vi "test Remote IO DIO Loop Back.vi"(8 "error in (no error)":errorcluster, 11 "TestCase in":refnum<class "Scan Engine EtherCAT System Tests.lvclass">) -> (0 "error out":errorcluster, 3 "TestCase out":refnum<class "Scan Engine EtherCAT System Tests.lvclass">)   [LabVIEW 2020, in "Scan Engine EtherCAT System Tests.lvclass"]
uses:
  Scan Engine EtherCAT System Tests.lvclass
  C:/Program Files (x86)/National Instruments/LabVIEW 2020/vi.lib/NI/VeriStand Custom Device Testing Tools/VeriStandTestCase/VeriStandTestCase.lvclass
  <vilib>/addons/_JKI Toolkits/VI Tester/TestCase.llb/TestCase.lvclass
  <vilib>/NI/VeriStand Custom Device Testing Tools/VeriStandTestCase/VeriStandTestCase.lvclass
  C:/Program Files (x86)/National Instruments/LabVIEW 2020/vi.lib/addons/_JKI Toolkits/VI Tester/TestCase.llb/TestCase.lvclass
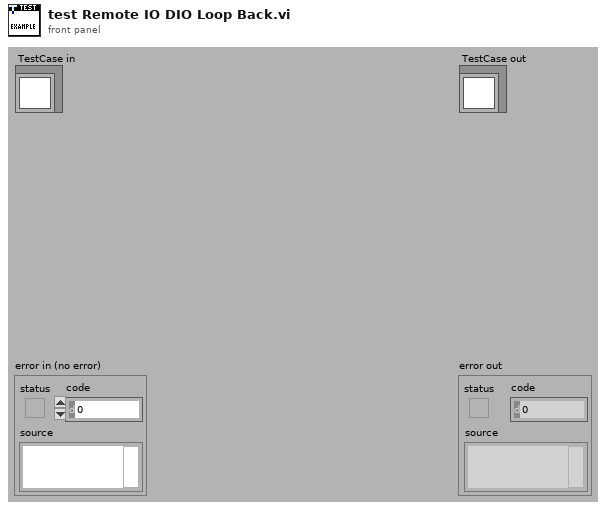
[diagram p1: front panel]
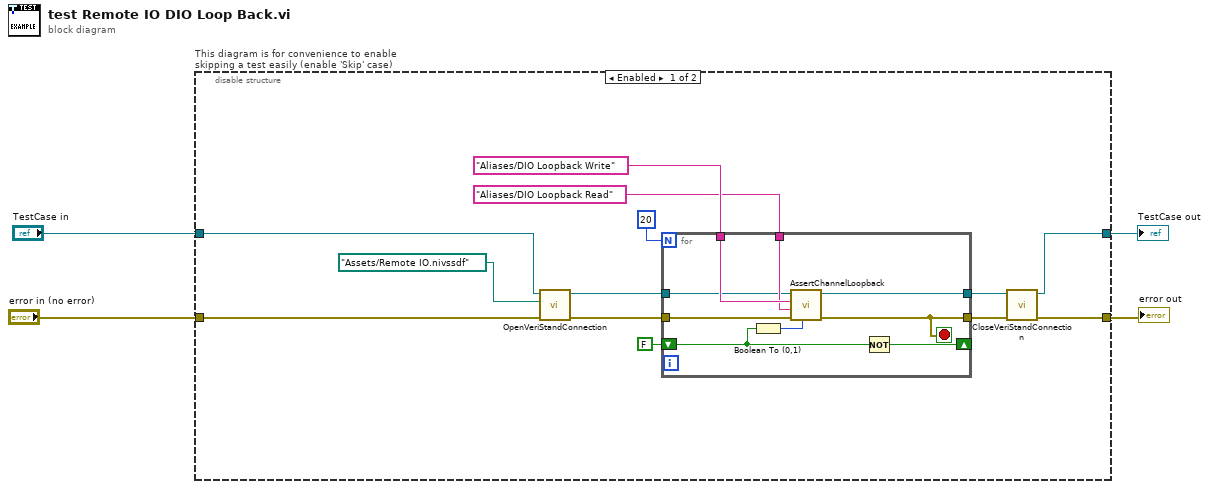
[diagram p0: block diagram]
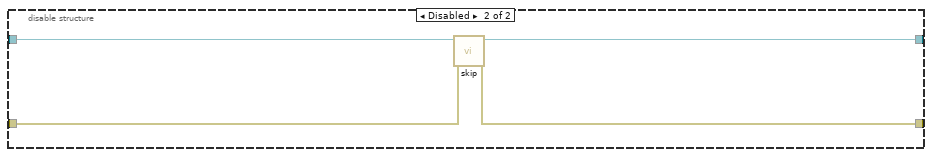
[diagram p2: hidden frame]
diagram:
  n1 = disable-structure "This diagram is for convenience to enable skipping a test easily (enable 'Skip' case)" shown="Enabled" {
    disable-tunnel: "TestCase in" -> [w6 w30]
    disable-tunnel: [w5 w28] -> w1
    disable-tunnel: [w8 w29] -> w3
    disable-tunnel: "error in (no error)" -> [w7 w27]
    frame Enabled {
      n2 = call-dynamic "OpenVeriStandConnection.vi"("error in (no error)"=w7, "System Definition File"=path "Assets/Remote IO.nivssdf", "VeriStand Test Case in"=w6) -> ("error out"=w12:errorcluster, "VeriStand Test Case out"=w11:refnum<class "Scan Engine EtherCAT System Tests.lvclass">)  [unwired: 6 in, 1 out]
      n3 = for {
        N: 20 -> [_]
        tunnel: "Aliases/DIO Loopback Write" ("Channel") -> [w23]
        tunnel: [w21] -> w10
        tunnel: "Aliases/DIO Loopback Read" ("Channel") -> [w22]
        shift-right: [w26] -> _
        shift-left: FALSE -> [w25]
        tunnel: w12 -> [w24]
        tunnel: [w18] -> w9
        tunnel: w11 -> [w19]
        stop <- w21 stop-if-true
        n4 = Boolean To (0,1)(Boolean=w25) -> (0, 1=w20:i16)
        n5 = call <vilib>:"AssertChannelLoopback.vi"("Value"=w20, "error in (no error)"=w24, "Read Channel"=w22, "Write Channel"=w23, "VeriStand Test Case in"=w19) -> ("error out"=w21:errorcluster, "VeriStand Test Case out"=w18:refnum<class "Scan Engine EtherCAT System Tests.lvclass">)  [unwired: 5 in]
        n6 = Not(x=w25) -> (.not. x?=w26:bool)
      }
      n7 = call-dynamic "CloseVeriStandConnection.vi"("error in (no error)"=w10, "VeriStand Test Case in"=w9) -> ("error out"=w8:errorcluster, "VeriStand Test Case out"=w5:refnum<class "Scan Engine EtherCAT System Tests.lvclass">)  [unwired: 8 in]
    }
    frame Disabled {
      n8 = call <vilib>:"skip.vi"("error in (no error)"=w27, "TestCase in"=w30) -> ("error out"=w29:errorcluster, "TestCase out"=w28:refnum<class "Scan Engine EtherCAT System Tests.lvclass">)  [unwired: 8 in]
    }
  }
  "error out" <- w3
  "TestCase out" <- w1
